vi "AfterPage2_GenCDP.vi"(10 "MetaDataObj":refnum<class "MetaDataObj.lvclass">, 11 "User Project":refnum<vi>) -> ()   [LabVIEW 2026, in "NIVS_CDEW_MetaDataObj.lvclass"]
uses:
  NIVS_CDEW_MetaDataObj.lvclass
  <resource>/dialog/NewProjectWizard/MetaDataObj/MetaDataObj.lvclass
  C:/Program Files/National Instruments/LabVIEW 2026/resource/dialog/NewProjectWizard/MetaDataObj/MetaDataObj.lvclass
  <resource>/dialog/NewProjectWizard/MetaDataObj/MetaDataObj.lvclass/MetaDataObj.ctl
  <resource>/dialog/NewProjectWizard/MetaDataObj/Accessors/Read Project Root.vi
  <resource>/dialog/NewProjectWizard/MetaDataObj/Accessors/Read Project Name.vi
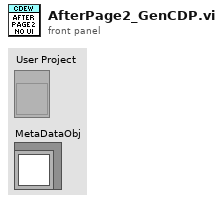
[diagram p1: front panel]
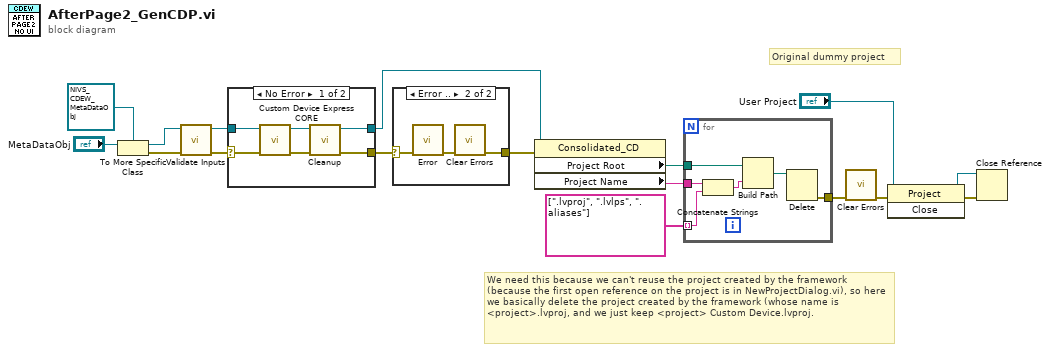
[diagram p0: block diagram]
diagram:
  # "Original dummy project"
  # "We need this because we can't reuse the project created by the framework (because the first open reference on the project is in NewProjectDialog.vi), so here we basically delete the project created by the framework (whose name is <project>.lvproj, and we just keep <project> Custom Device.lvproj."
  n1 = To More Specific Class(target class=refnum<class "NIVS_CDEW_MetaDataObj.lvclass"> refnum ("NIVS_CDW_MetaDataObj.lvclass"), reference="MetaDataObj") -> (specific class reference=w2:refnum<class "NIVS_CDEW_MetaDataObj.lvclass">, error out=w6:errorcluster)  [unwired: 1 in]
  n2 = call "Validate Inputs.vi"("error in"=w6, "CDPW_MetaDataObj"=w2) -> ("error out"=w4:errorcluster, "CDPW_MetaDataObj"=w5:refnum<class "NIVS_CDEW_MetaDataObj.lvclass">)  [unwired: 8 in]
  n3 = case shown="No Error" w4 {
    selector: w4 -> [w22 w25]
    tunnel: [w18 w25] -> w3
    tunnel: w5 -> [w23 w24]
    tunnel: [w19 w24] -> w1
    frame No Error {
      n4 = call "Custom Device Express CORE.vi"("error in"=w22, "CDEW_MetaDataObj in"=w23) -> ("error out"=w20:errorcluster, "CDEW_MetaDataObj out"=w21:refnum<class "NIVS_CDEW_MetaDataObj.lvclass">)  [unwired: 8 in]
      n5 = call "Cleanup.vi"("error in"=w20, "Consolidated_CD in"=w21) -> ("error out"=w18:errorcluster, "Consolidated_CD out"=w19:refnum<class "NIVS_CDEW_MetaDataObj.lvclass">)  [unwired: 8 in]
    }
    frame Error {
    }
  }
  n6 = case shown="Error .." w3 {
    selector: w3 -> [w26 w28]
    tunnel: [w26 w29] -> w8
    frame No Error {
    }
    frame Error {
      n7 = call "Error.vi"("error in"=w28) -> ("error out"=w27:errorcluster)  [unwired: 10 in]
      n8 = call <vilib>:"Clear Errors.vi"("error in (no error)"=w27) -> ("error out"=w29:errorcluster)  [unwired: 5 in, 1 out]
    }
  }
  n9 = property class="Consolidated_CD"(reference=w1, error in=w8) -> ("Project Root"=w16:path, "Project Name"=w15:string)  [unwired: 2 out]
  n10 = for {
    tunnel: w16 -> [w35]
    tunnel: w15 -> [w34]
    tunnel: string[] [".lvproj", ".lvlps", ".aliases"] -> [w33] mode=indexing
    tunnel: [w30] -> w13
    n11 = Concatenate Strings(w34, w33) -> (w32:string)
    n12 = Build Path(base path=w35, name or relative path=w32) -> (appended path=w31:path)
    n13 = Delete(path (use dialog)=w31) -> (error out=w30:errorcluster)  [unwired: 4 in, 2 out]
  }
  n14 = call <vilib>:"Clear Errors.vi"("error in (no error)"=w13) -> ("error out"=w12:errorcluster)  [unwired: 5 in, 1 out]
  n15 = invoke class="Project" method="Close"(reference="User Project", error in=w12) -> (reference out=w9:refnum<vi>, error out=w10:errorcluster)  [unwired: 1 in, 1 out]
  n16 = Close Reference(reference=w9, error in (no error)=w10) -> ()  [unwired: 1 out]
